vi "Postgresql Connect.vi"(8 "error in (no error)":errorcluster, 10 "Connection String":string, 11 "PGJDPMapper":refnum<class "Mapper.lvclass">) -> (0 "error out":errorcluster, 3 "SqlMapper out":refnum<class "SqlMapper.lvclass">)   [LabVIEW 2020, in "ORM_pgsql_jdp.lvlib" / "DBC.lvclass"]
uses:
  DBC.lvclass
  DBC.lvclass/DBC.ctl
  <vilib>/Viviota/shared/ORM.lvlibp/SqlMapper/SqlMapper.lvclass
  PGJDPMapper/Mapper.lvclass
  C:/Program Files/National Instruments/LabVIEW 2020/vi.lib/Viviota/shared/ORM.lvlibp/SqlMapper/SqlMapper.lvclass
  C:/Program Files/National Instruments/LabVIEW 2020/vi.lib/Viviota/shared/ORM.lvlibp/DbConnection/DbConnection.lvclass
  C:/Viviota/Projects/R&D/__OpenSource/labview-orm/DirectConnections/pgsql_jdp/dbc/DBC.lvclass
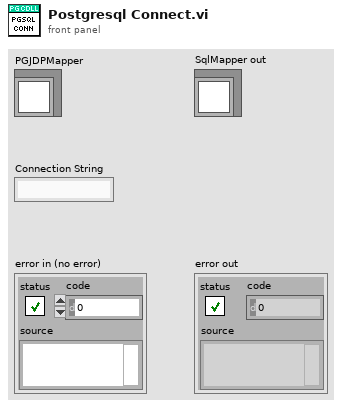
[diagram p1: front panel]
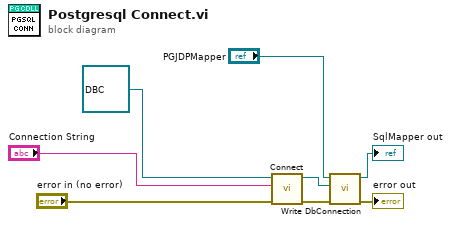
[diagram p0: block diagram]
diagram:
  n1 = call-dynamic "Connect.vi"("error in (no error)"="error in (no error)", "Connection String"="Connection String", "PostgresqlConnection in"=refnum<class "DBC.lvclass"> refnum ("PostgresqlConnection.lvclass")) -> ("error out"=w5:errorcluster, "PostgresqlConnection out"=w3:refnum<class "DBC.lvclass">)  [unwired: 7 in]
  n2 = call <vilib>:"Write DbConnection.vi"("error in (no error)"=w5, "Dapper.lvlib:DbConnection.lvclass"=w3, "SqlMapper in"="PGJDPMapper") -> ("error out"=→"error out":errorcluster, "SqlMapper out"=→"SqlMapper out":refnum<class "Mapper.lvclass">)  [unwired: 7 in]
